vi "onLock.vi"(8 "error in (no error)":errorcluster, 10 "Player":refnum<class "Player.lvclass">, 11 "LockedState in":refnum<class "LockedState.lvclass">) -> (0 "error out":errorcluster, 1 "String":string, 2 "Player out":refnum<class "Player.lvclass">, 3 "LockedState out":refnum<class "LockedState.lvclass">)   [LabVIEW 2018, in "LockedState.lvclass"]
uses:
  LockedState.lvclass
  Player Class/Player.lvclass
  Player Class/Player.lvclass/Player.ctl
  ReadyState Class/ReadyState.lvclass
  C:/Users/fflores/Documents/LabVIEW-Open-Projects/LabIVEW OOP Design Patterns/State Pattern/State Class/State.lvclass
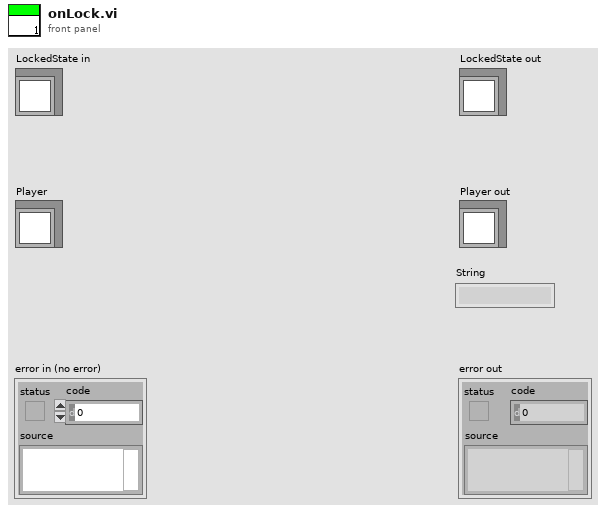
[diagram p1: front panel]
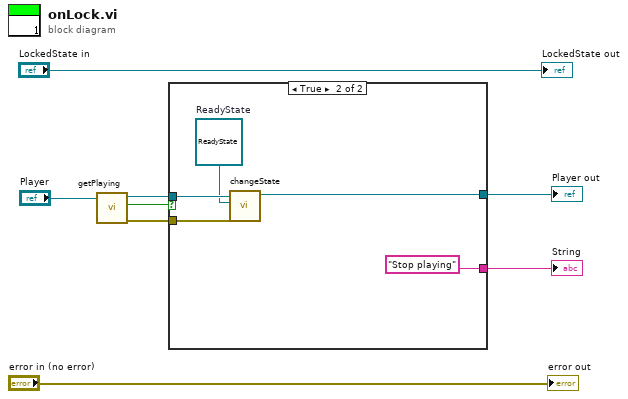
[diagram p0: block diagram]
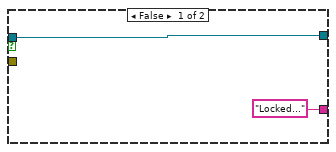
[diagram p2: hidden frame]
diagram:
  n1 = call "getPlaying.vi"("Player in"="Player") -> ("error out"=w4:errorcluster, "playing"=w2:bool, "Player out"=w3:refnum<class "Player.lvclass">)  [unwired: 8 in]
  n2 = case shown="True" w2 {
    tunnel: ["Locked..." "Stop playing"] -> w5
    tunnel: w4 -> [_ w14]
    tunnel: w3 -> [w9 w13]
    tunnel: [w9 w11] -> w1
    frame False {
    }
    frame True {
      w12 = refnum<class "ReadyState.lvclass"> refnum  # ReadyState
      n3 = call-dynamic "changeState.vi"("error in (no error)"=w14, "State"=w12, "Player in"=w13) -> ("Player out"=w11:refnum<class "Player.lvclass">)  [unwired: 7 in, 1 out]
    }
  }
  "String" <- w5
  "Player out" <- w1
  "error out" <- "error in (no error)"
  "LockedState out" <- "LockedState in"
